vi "test_Multiple Writes and Reads.vi"(8 "error in (no error)":errorcluster, 11 "Scalar Channels Testing in":refnum<class "FPGA Addon Scalar Channels System Tests.lvclass">) -> (0 "error out":errorcluster, 3 "Scalar Channels Testing out":refnum<class "FPGA Addon Scalar Channels System Tests.lvclass">)   [LabVIEW 2020, in "FPGA Addon Scalar Channels System Tests.lvclass"]
uses:
  FPGA Addon Scalar Channels System Tests.lvclass
  C:/Users/nitest/Desktop/Git 2020/niveristand-fpga-addon-custom-device/Source/Tests/FPGA Addon Test Class/FPGA Addon Test Class.lvclass
  C:/Program Files (x86)/National Instruments/LabVIEW 2020/vi.lib/NI/VeriStand Custom Device Testing Tools/VeriStandTestCase/VeriStandTestCase.lvclass
  FPGA Addon Test Class/FPGA Addon Test Class.lvclass/FPGA Addon Test Class.ctl
  FPGA Addon Test Class/FPGA Addon Test Class.lvclass
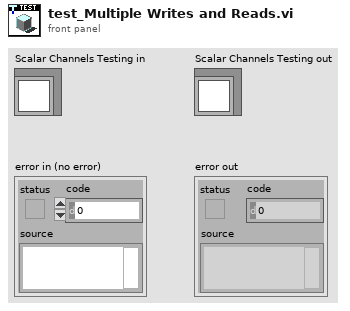
[diagram p1: front panel]
types:
  T1 = typedef "NI_VS Workspace ExecutionAPI.lvlib/WorkspaceAPI.ctl" = refnum<k24>
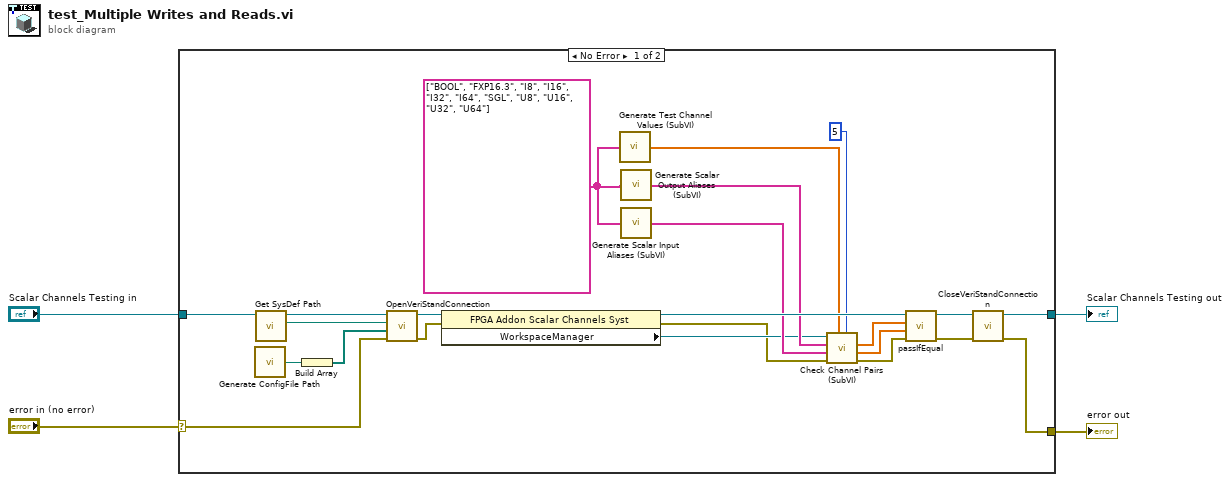
[diagram p0: block diagram]
diagram:
  n1 = case shown="No Error" "error in (no error)" {
    selector: "error in (no error)" -> [w20 w29]
    tunnel: [w26 w29] -> w3
    tunnel: [w27 w28] -> w1
    tunnel: "Scalar Channels Testing in" -> [w10 w28]
    frame No Error {
      w15 = string[] ["BOOL", "FXP16.3", "I8", "I16", "I32", "I64", "SGL", "U8", "U16", "U32", "U64"]
      n2 = call "Generate ConfigFile Path.vi"() -> ("ConfigFile path"=w7:path)
      n3 = call "Get SysDef Path.vi"("Scalar Channels Testing in"=w10) -> ("SysDef Path"=w8:path, "Scalar Channels Testing out"=w9:refnum<class "FPGA Addon Scalar Channels System Tests.lvclass">)  [unwired: 9 in]
      n4 = Build Array(w7) -> (w6:path[])
      n5 = call-dynamic "OpenVeriStandConnection.vi"("error in (no error)"=w20, "overrides files"=w6, "System Definition File"=w8, "VeriStand Test Case in"=w9) -> ("error out"=w25:errorcluster, "VeriStand Test Case out"=w24:refnum<class "FPGA Addon Scalar Channels System Tests.lvclass">)  [unwired: 5 in, 1 out]
      n6 = property class="FPGA Addon Scalar Channels Syst"(reference=w24, error in=w25) -> (reference out=w22:refnum<class "FPGA Addon Scalar Channels System Tests.lvclass">, error out=w11:errorcluster, "WorkspaceManager"=w12:T1)
      n7 = call "Generate Test Channel Values (SubVI).vi"("Aliases in"=w15) -> ("Test Channel Values out"=w17:dbl[])
      n8 = call "Generate Scalar Output Aliases (SubVI).vi"("Aliases Seed"=w15) -> ("Scalar Output Aliases"=w14:string[])
      n9 = call "Generate Scalar Input Aliases (SubVI).vi"("Aliases Seed"=w15) -> ("Scalar Input Aliases"=w13:string[])
      n10 = call "Check Channel Pairs (SubVI).vi"("seconds to wait"=u32 5 ("milliseconds to wait"), "Test Values"=w17, "error in (no error)"=w11, "Scalar Input Aliases"=w13, "Scalar Output Aliases"=w14, ".NET Refnum in"=w12) -> ("error out"=w5:errorcluster, "Input Scalar Channel Values"=w18:dbl[], "Output Scalar Channel Values"=w19:dbl[])  [unwired: 2 in, 1 out]
      n11 = call-dynamic "passIfEqual.vi"("error in (no error)"=w5, "y"=w18, "x"=w19, "TestCase in"=w22) -> ("error out"=w23:errorcluster, "TestCase out"=w21:refnum<class "FPGA Addon Scalar Channels System Tests.lvclass">)  [unwired: 6 in]
      n12 = call-dynamic "CloseVeriStandConnection.vi"("error in (no error)"=w23, "VeriStand Test Case in"=w21) -> ("error out"=w26:errorcluster, "VeriStand Test Case out"=w27:refnum<class "FPGA Addon Scalar Channels System Tests.lvclass">)  [unwired: 8 in]
    }
    frame Error {
    }
  }
  "error out" <- w3
  "Scalar Channels Testing out" <- w1
